vi "clock gauge.vi"() -> ()   [LabVIEW 2016]
panel:
  in  "Numeric":i32=120
  out "Gauge":dbl(knob) scale=0.0..60.0
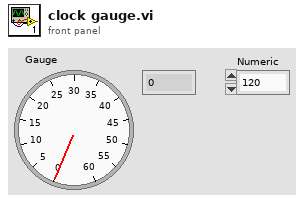
[diagram p1: front panel]
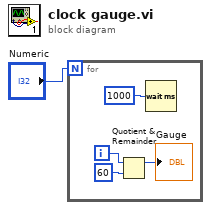
[diagram p0: block diagram]
diagram:
  n1 = for {
    N: "Numeric" -> [_]
    i -> [w4]
    n2 = Quotient & Remainder(x=w4, y=60) -> (x-y*floor(x/y)=→"Gauge":i32)  [unwired: 1 out]
    n3 = Wait (ms)(milliseconds to wait=u32 1000) -> ()  [unwired: 1 out]
  }
